vi "Convert LIN frames to Trace log.vi"(11 "lin frames in":T1[](array[typedef]) {"event ID" format="%x"; "payload" format="%x"; "timestamp" format="%<%.7X\n%x>T"; "type" items=["LIN Data"=64, "LIN Bus Error"=65, "LIN No Response"=66, "Delay"=224, "Log Trigger"=225, "Start Trigger"=226]; "identifier" format="%x"}) -> (3 "trace out":string[][](array[string]))   [LabVIEW 2025, in "CAN-LIN Raw Bus Capture.lvclass"]
uses:
  CAN-LIN Raw Bus Capture.lvclass
  <vilib>/xnet/xnet.llb/XNET Frame LIN.ctl
  <vilib>/xnet/xnet.llb/XNET Frame Type LIN.ctl
  CAN-LIN Raw Bus Capture.lvclass/CAN-LIN Raw Bus Capture.ctl
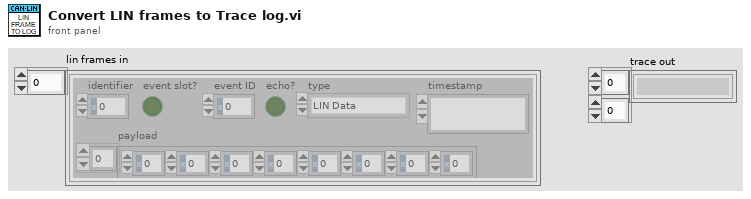
[diagram p1: front panel]
types:
  T1 = typedef "XNET Frame LIN.ctl" = cluster{"timestamp":timestamp, "payload":u8[], "identifier":u32, "type":T2, "event ID":u8, "event slot?":bool, "echo?":bool}
  T2 = typedef "XNET Frame Type LIN.ctl" = u8
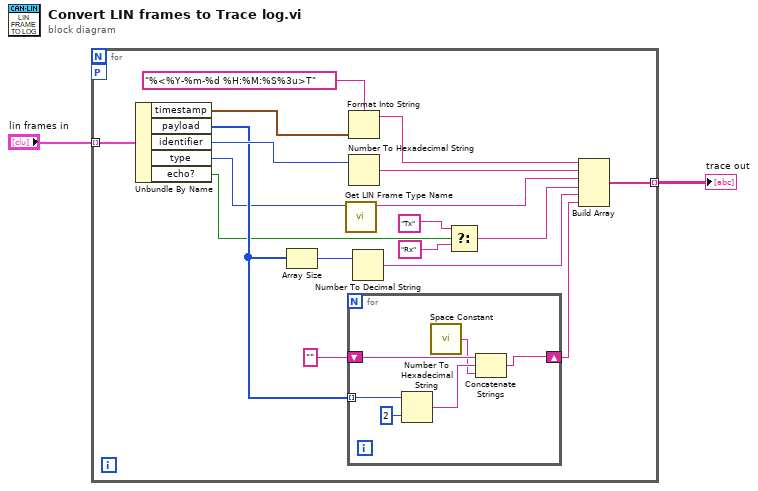
[diagram p0: block diagram]
diagram:
  n1 = for {
    tunnel: "lin frames in" -> [w20] mode=indexing
    tunnel: [w17] -> w2 mode=indexing
    workers-P: _ -> [_]
    n2 = Unbundle By Name(w20) -> ("timestamp"=w16:timestamp, "payload"=w12:u8[], "identifier"=w19:u32, "type"=w10:T2, "echo?"=w4:bool)
    n3 = Array Size(array=w12) -> (size(s)=w13:i32)
    n4 = call "Get LIN Frame Type Name.vi"("lin frame type id"=w10) -> ("lin frame type name"=w9:string)  [unwired: 10 in]
    n5 = for {
      tunnel: w12 -> [w26] mode=indexing
      shift-right: [w23] -> w8
      shift-left: "" ("format string") -> [w25]
      n6 = Number To Hexadecimal String(1:i16 2 ("width (-)"), 2:w26) -> (0:w24:string)
      n7 = call <vilib>:"Space Constant.vi"() -> ("String"=w21:string)
      n8 = Concatenate Strings(w25, w24, w21) -> (w23:string)
    }
    n9 = Format Into String(format string="%<%Y-%m-%d %H:%M:%S%3u>T", w16) -> (resulting string=w15:string)  [unwired: 2 in, 1 out]
    n10 = Number To Hexadecimal String(2:w19) -> (0:w18:string)  [unwired: 1 in]
    n11 = Number To Decimal String(number=w13) -> (decimal integer string=w7:string)  [unwired: 1 in]
    n12 = Select(t="Tx" ("format string"), s=w4, f="Rx" ("format string")) -> (s? t:f=w3:string)
    n13 = Build Array(w15, w18, w9, w3, w7, w8) -> (w17:string[])
  }
  "trace out" <- w2
